vi "2_VI_Auto.vi"   [LabVIEW 2024]
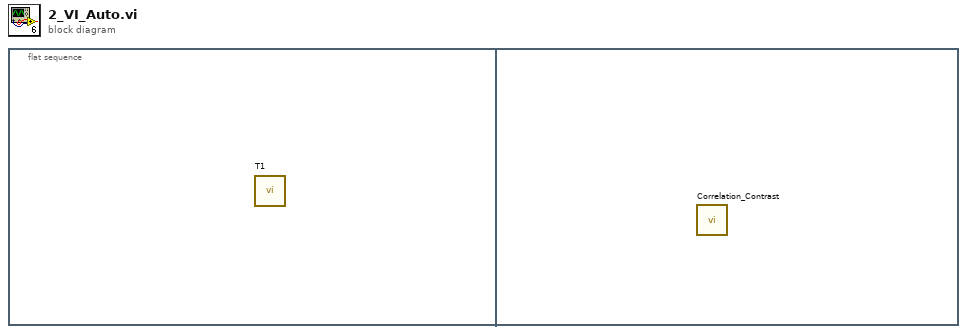
[diagram p0: block diagram]
diagram:
  n1 = flat-sequence {
    frame #0 {
      n2 = call "T1.vi"() -> ()  [unwired: 12 in]
    }
    frame #1 {
      n3 = call "Correlation_Contrast.vi"() -> ()  [unwired: 12 in]
    }
  }
